vi "Insert Into TreeView.vi"(7 "Path delimiter (/)":string="/", 8 "error in (no error)":errorcluster, 9 "Item values":string[](array[string]), 10 "Item path":string, 11 "TreeControl Ref":refnum<vi>) -> (0 "error out":errorcluster, 3 "TreeControl Ref Out":refnum<vi>)   [LabVIEW 2019]
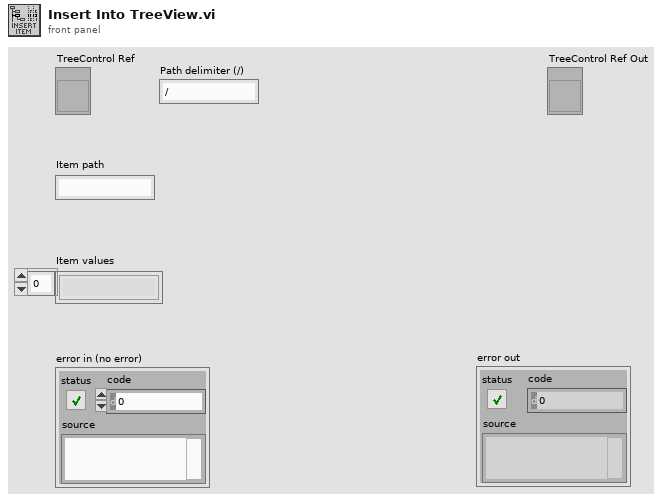
[diagram p1: front panel]
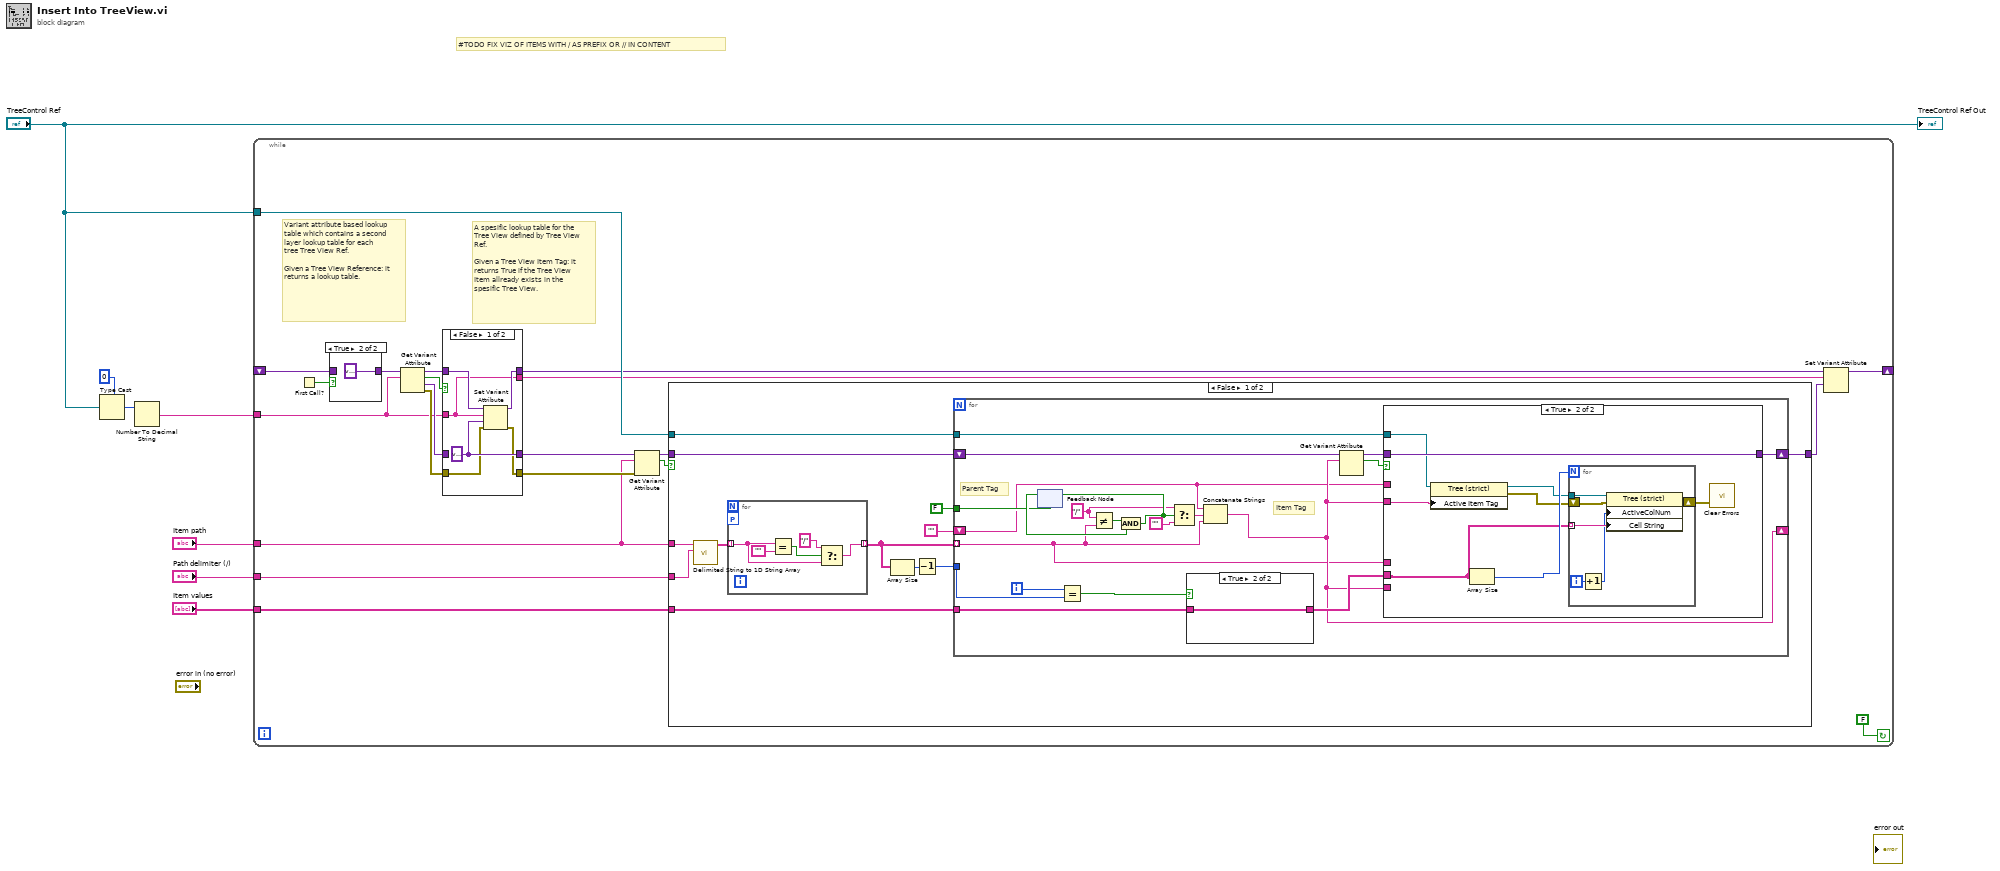
[diagram p0: block diagram]
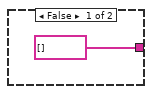
[diagram p2: hidden frame]
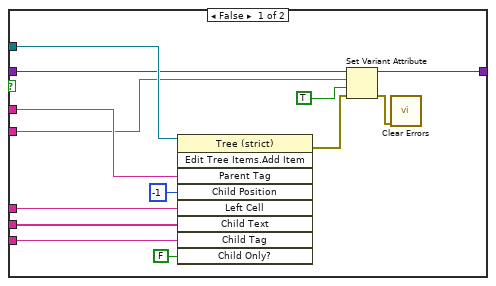
[diagram p3: hidden frame]
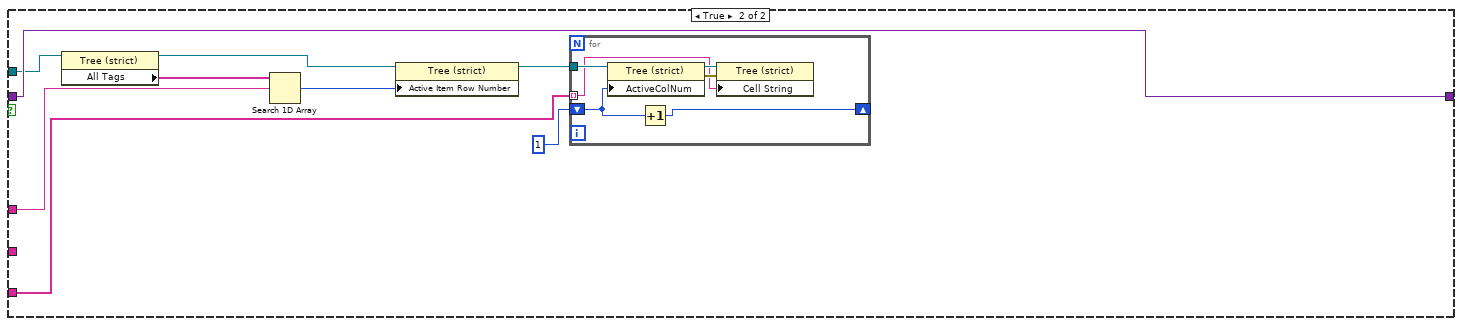
[diagram p4: hidden frame]
diagram:
  # "#TODO FIX VIZ OF ITEMS WITH / AS PREFIX OR // IN CONTENT"
  n1 = Type Cast(type=u64 0, x="TreeControl Ref") -> (*(type *) &x=w3:u64)
  n2 = Number To Decimal String(number=w3) -> (decimal integer string=w2:string)  [unwired: 1 in]
  n3 = while {
    shift-right: [w15] -> _
    shift-left: _ -> [w27]
    tunnel: "Item path" -> [w8]
    tunnel: "Item values" -> [w19]
    tunnel: "TreeControl Ref" -> [w18]
    tunnel: w2 -> [w10]
    tunnel: "Path delimiter (/)" -> [w9]
    stop <- FALSE continue-if-true
    # "A spesific lookup table for the Tree View defined by Tree View Ref.\n\nGiven a Tree View Item Tag: it returns True if the Tree View Item allready exists in the spesific Tree View."
    # "Variant attribute based lookup table which contains a second layer lookup table for each tree Tree View Ref.\n\nGiven a Tree View Reference: it returns a lookup table."
    n4 = First Call?() -> (First Call?: T/F=w28:bool)
    n5 = case shown="True" w28 {
      tunnel: w27 -> [w120 _]
      tunnel: [w120 variant ("variant")] -> w26
      frame False {
      }
      frame True {
      }
    }
    n6 = Get Variant Attribute(Variant=w26, name=w10) -> (duplicate Variant=w24:variant, found=w25:bool, value=w23:variant, error out=w12:errorcluster)  [unwired: 2 in]
    n7 = case shown="False" w25 {
      tunnel: w24 -> [w115 w119]
      tunnel: [w114 w119] -> w16
      tunnel: [w113 w118] -> w22
      tunnel: w23 -> [_ w118]
      tunnel: w10 -> [w112 w117]
      tunnel: [w112 w117] -> w13
      tunnel: w12 -> [w110 w116]
      tunnel: [w111 w116] -> w11
      frame False {
        w113 = variant ("variant")
        n8 = Set Variant Attribute(Variant=w115, name=w112, value=w113, error in=w110) -> (Variant out=w114:variant, error out=w111:errorcluster)  [unwired: 1 out]
      }
      frame True {
      }
    }
    n9 = Get Variant Attribute(Variant=w22, name=w8, error in=w11) -> (duplicate Variant=w20:variant, found=w21:bool)  [unwired: 1 in, 2 out]
    n10 = case shown="False" w21 {
      tunnel: w20 -> [w39 w103]
      tunnel: w8 -> [w40 w96]
      tunnel: w19 -> [w36 w99]
      tunnel: w18 -> [w38 w101]
      tunnel: [w35 w103] -> w14
      tunnel: w9 -> [w32 _]
      frame False {
        n11 = call <vilib>:"Delimited String to 1D String Array.vi"("delimiter"=w32, "delimited string"=w40) -> ("string array"=w31:string[])  [unwired: 9 in]
        n12 = for {
          tunnel: w31 -> [w42] mode=indexing
          tunnel: [w41] -> w30 mode=indexing
          workers-P: _ -> [_]
          n13 = Equal?(x=w42, y="") -> (x = y?=w44:bool)
          n14 = Select(t="/", s=w44, f=w42) -> (s? t:f=w41:string)
        }
        n15 = Array Size(array=w30) -> (size(s)=w34:i32)
        n16 = Decrement(x=w34) -> (x-1=w33:i32)
        n17 = for {
          tunnel: w30 -> [w47] mode=indexing
          tunnel: w38 -> [w63]
          shift-right: [w52] -> _
          shift-left: "" -> [w46]
          tunnel: w36 -> [w62]
          shift-right: [w59] -> w35
          shift-left: w39 -> [w65]
          tunnel: w33 -> [w58]
          tunnel: FALSE -> [w49]
          i -> [w56]
          w48 = "/"
          # "Item Tag"
          # "Parent Tag"
          n18 = feedback #1(w49) -> (w50:bool)
          n19 = Equal?(x=w56, y=w58) -> (x = y?=w57:bool)
          n20 = Not Equal?(x=w48, y=w47) -> (x != y?=w55:bool)
          n21 = And(x=w55, y=w50) -> (x .and. y?=w51:bool)
          n22 = feedback-in #1(w51) -> ()
          n23 = Select(t=w48, s=w51, f="") -> (s? t:f=w53:string)
          n24 = case shown="True" w57 {
            tunnel: w62 -> [_ w67]
            tunnel: [string[] [] ("Values") w67] -> w61
            frame False {
            }
            frame True {
            }
          }
          n25 = Concatenate Strings(w46, w53, w47) -> (w52:string)
          n26 = Get Variant Attribute(Variant=w65, name=w52) -> (duplicate Variant=w60:variant, found=w64:bool)  [unwired: 2 in, 2 out]
          n27 = case shown="True" w64 {
            tunnel: w63 -> [w80 w87]
            tunnel: w52 -> [w79 _]
            tunnel: w46 -> [w78 _]
            tunnel: w47 -> [w75 _]
            tunnel: w61 -> [w77 w84]
            tunnel: w60 -> [w76 w88]
            tunnel: [w74 w88] -> w59
            tunnel: w52 -> [w72 w86]
            frame False {
              n28 = invoke class="Tree (strict)" method="Edit Tree Items.Add Item"(reference=w80, "Parent Tag"=w78, "Child Position"=-1, "Left Cell"=w75, "Child Text"=w77, "Child Tag"=w79, "Child Only?"=FALSE) -> (error out=w70:errorcluster)  [unwired: 2 in, 8 out]
              n29 = Set Variant Attribute(Variant=w76, name=w72, value=TRUE, error in=w70) -> (Variant out=w74:variant, error out=w68:errorcluster)  [unwired: 1 out]
              n30 = call <vilib>:"Clear Errors.vi"("error in (no error)"=w68) -> ()  [unwired: 5 in, 2 out]
            }
            frame True {
              n31 = property class="Tree (strict)"(reference=w87, "Active Item Tag"=w86) -> (reference out=w83:refnum<vi>, error out=w82:errorcluster)  [unwired: 1 in]
              n32 = Array Size(array=w84) -> (size(s)=w85:i32)
              n33 = for {
                N: w85 -> [_]
                tunnel: w84 -> [w93] mode=indexing
                tunnel: w83 -> [w92]
                shift-right: [w89] -> w81
                shift-left: w82 -> [w90]
                i -> [w94]
                n34 = Increment(x=w94) -> (x+1=w91:i32)
                n35 = property class="Tree (strict)"(reference=w92, error in=w90, "ActiveColNum"=w91, "Cell String"=w93) -> (error out=w89:errorcluster)  [unwired: 1 out]
              }
              n36 = call <vilib>:"Clear Errors.vi"("error in (no error)"=w81) -> ()  [unwired: 5 in, 2 out]
            }
          }
        }
      }
      frame True {
        n37 = property class="Tree (strict)"(reference=w101) -> (reference out=w100:refnum<vi>, "All Tags"=w97:string[])  [unwired: 1 in, 1 out]
        n38 = Search 1D Array(1D array=w97, element=w96) -> (index of element=w95:i32)  [unwired: 1 in]
        n39 = property class="Tree (strict)"(reference=w100, "Active Item Row Number"=w95) -> (reference out=w102:refnum<vi>)  [unwired: 1 in, 1 out]
        n40 = for {
          tunnel: w102 -> [w109]
          tunnel: w99 -> [w106] mode=indexing
          shift-right: [w105] -> _
          shift-left: 1 -> [w104]
          n41 = property class="Tree (strict)"(reference=w109, "ActiveColNum"=w104) -> (reference out=w108:refnum<vi>, error out=w107:errorcluster)  [unwired: 1 in]
          n42 = Increment(x=w104) -> (x+1=w105:i32)
          n43 = property class="Tree (strict)"(reference=w108, error in=w107, "Cell String"=w106) -> ()  [unwired: 2 out]
        }
      }
    }
    n44 = Set Variant Attribute(Variant=w16, name=w13, value=w14) -> (Variant out=w15:variant)  [unwired: 1 in, 2 out]
  }
  "TreeControl Ref Out" <- "TreeControl Ref"
